vi "LabVIEWStatus.vi"(9 "Mode XML Elements":string, 11 "License Information":refnum<vi>) -> (3 "License Status Text":string)   [LabVIEW 2023, in "GettingStartedWindow.lvlib"]
uses:
  <resource>/modes/FRC/GettingStartedWindow.lvlib
  <resource>/modes/FRC/LocalizedStrings.vi
  <vilib>/Utility/miscctls.llb/LVPositionTypeDef.ctl
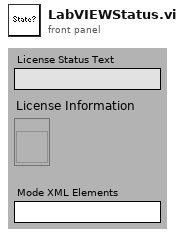
[diagram p1: front panel]
types:
  T1 = typedef "LVPositionTypeDef.ctl" = cluster{"Left":i32, "Top":i32}
  T2 = enum32{"invalid OS target", "Mac OS", "Windows 3.1", "Windows 95/NT", "Solaris 1", "Solaris 2", "HP-UX", "PowerMAX", "Linux", "Irix", "Rhapsody", "BeOS", "AIX", "OSF1", "VxWorks", "PharLap", "Carbon", "RTX", "Windows x64", "Linux x64", "Mac OS X x64", "Windows ARM64", "Linux ARM64", "Mac OS X ARM64"}
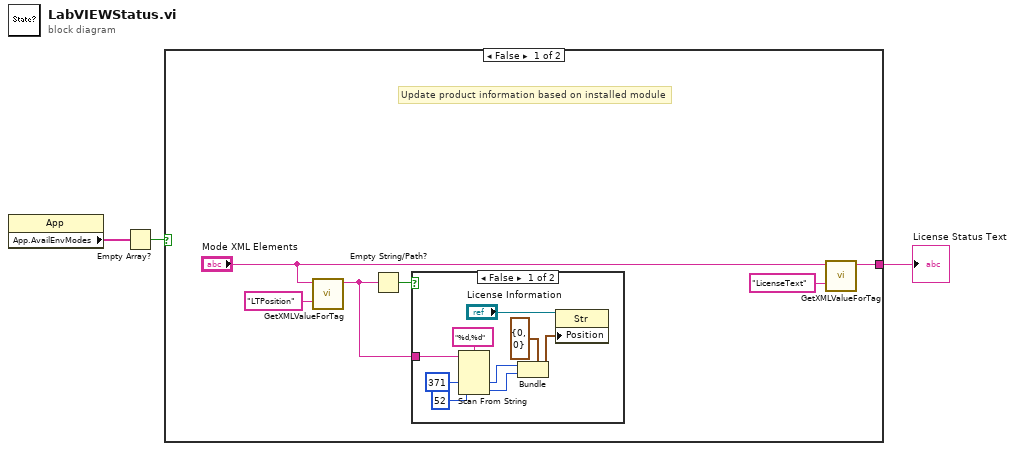
[diagram p0: block diagram]
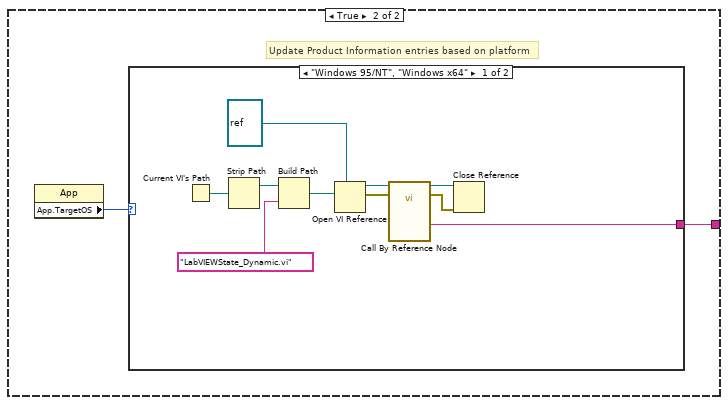
[diagram p3: hidden frame]
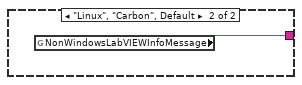
[diagram p4: hidden frame]
diagram:
  n1 = property class="App"() -> ("App.AvailEnvModes"=w1:string[])  [unwired: 2 in, 2 out]
  n2 = Empty Array?(array=w1) -> (empty?=w2:bool)
  n3 = case shown="False" w2 {
    tunnel: [w8 w19] -> w3
    frame False {
      # "Update product information based on installed module"
      n4 = call <resource>:"GetXMLValueForTag.vi"("tag"="LTPosition" ("key"), "XML"="Mode XML Elements") -> ("value"=w4:string)  [unwired: 1 in, 8 out]
      n5 = Empty String/Path?(string/path=w4) -> (empty?=w5:bool)
      n6 = case shown="False" w5 {
        tunnel: w4 -> [w14 _]
        frame False {
          n7 = Scan From String(format string="%d,%d", input string=w14, default 1=371 ("default value 1"), default 2=52 ("default value 2")) -> (output 1=w13:i32, output 2=w12:i32)  [unwired: 2 in, 3 out]
          n8 = Bundle(cluster=T1 {"Left"=0, "Top"=0} ("Position"), "Left"=w13, "Top"=w12) -> (w10:T1)
          n9 = property class="Str"(reference="License Information", "Position"=w10) -> ()  [unwired: 1 in, 2 out]
        }
        frame True {
        }
      }
      n10 = call <resource>:"GetXMLValueForTag.vi"("tag"="LicenseText" ("key"), "XML"="Mode XML Elements") -> ("value"=w8:string)  [unwired: 1 in, 8 out]
    }
    frame True {
      # "Update Product Information entries based on platform"
      n11 = property on="Property Node" class="App"() -> ("App.TargetOS"=w20:T2)  [unwired: 2 in, 2 out]
      n12 = case shown="\"Windows 95/NT\", \"Windows x64\"" w20 {
        tunnel: [w21 w31] -> w19
        frame "Windows 95/NT", "Windows x64" {
          n13 = Current VI's Path() -> (path=w30:path)
          n14 = Strip Path(path=w30) -> (stripped path=w29:path)  [unwired: 1 out]
          n15 = Build Path(base path=w29, name or relative path="LabVIEWState_Dynamic.vi") -> (appended path=w27:path)
          n16 = Open VI Reference(type specifier VI Refnum (for type only)=refnum<vi> refnum ("VI Refnum"), vi path=w27) -> (vi reference=w24:refnum<vi>, error out=w26:errorcluster)  [unwired: 1 in, 3 out]
          n17 = call-by-ref "Call By Reference Node"(reference=w24, error in=w26) -> (reference out=w22:refnum<vi>, error out=w23:errorcluster, "LabVIEW State String"=w21:string)  [unwired: 10 in, 1 out]
          n18 = Close Reference(reference=w22, error in (no error)=w23) -> ()  [unwired: 1 out]
        }
        frame "Linux", "Carbon", Default {
          n19 = global read "LocalizedStrings.vi" "NonWindowsLabVIEWInfoMessage"() -> (w31:string)
        }
      }
    }
  }
  "License Status Text" <- w3
